vi "Run Tests.vi"(11 "Arguments":string[](array[string])) -> (2 "CLI Message":string, 3 "CLI Return Code":i32)   [LabVIEW 2026]
doc: "Caraya suite runner, generated by lvai_generate_caraya_test_runner.\n\nIt builds every test VI's path relative to its OWN location, so the suite moves with the folder, and runs them through Caraya's Run Tests.vi (Array Path instance) with Interactive FALSE - a TRUE there opens a modal report dialog, which stops LabVIEW's gRPC service until a human dismisses it.\n\nRead the JUnit report named by 'Report Path used', not 'error out': the error cluster carries the FIRST failed assertion only."
uses:
  <vilib>/addons/_JKI Toolkits/Caraya/run-tests/Run Test (Array Path).vi
  <vilib>/addons/_JKI Toolkits/Caraya/Caraya.lvlib
panel:
  out "error out":errorcluster
  out "Report Path used":path
  in  "error in":errorcluster
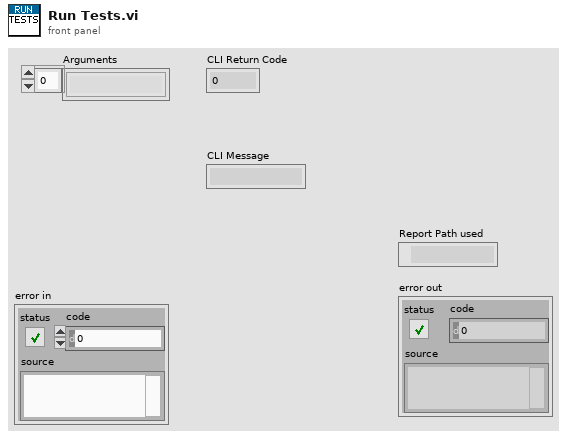
[diagram p1: front panel]
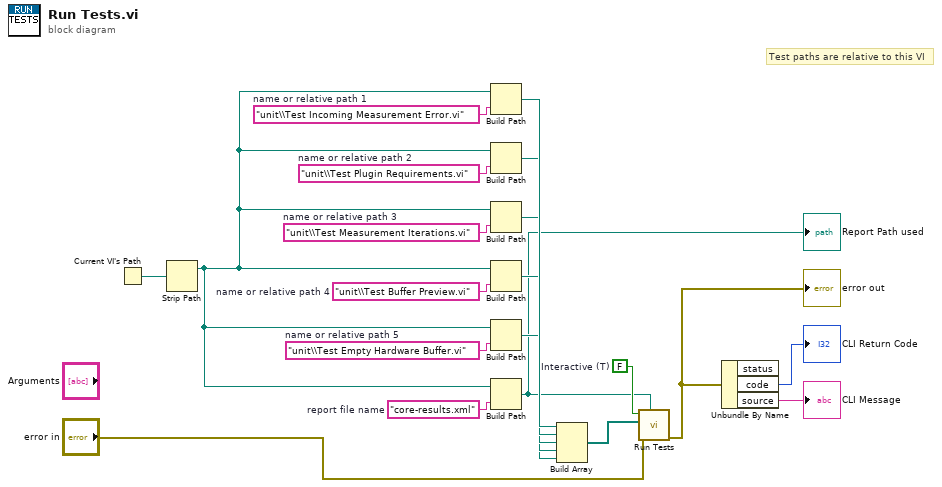
[diagram p0: block diagram]
diagram:
  w7 = FALSE  # Interactive (T)
  w13 = "core-results.xml"  # report file name
  w15 = "unit\\Test Empty Hardware Buffer.vi"  # name or relative path 5
  w16 = "unit\\Test Buffer Preview.vi"  # name or relative path 4
  w17 = "unit\\Test Measurement Iterations.vi"  # name or relative path 3
  w18 = "unit\\Test Plugin Requirements.vi"  # name or relative path 2
  w19 = "unit\\Test Incoming Measurement Error.vi"  # name or relative path 1
  # "Test paths are relative to this VI"
  n1 = Current VI's Path() -> (path=w20:path)
  n2 = Strip Path(path=w20) -> (stripped path=w14:path)  [unwired: 1 out]
  n3 = Build Path(base path=w14, name or relative path=w19) -> (appended path=w12:path)
  n4 = Build Path(base path=w14, name or relative path=w18) -> (appended path=w11:path)
  n5 = Build Path(base path=w14, name or relative path=w17) -> (appended path=w10:path)
  n6 = Build Path(base path=w14, name or relative path=w16) -> (appended path=w9:path)
  n7 = Build Path(base path=w14, name or relative path=w15) -> (appended path=w8:path)
  n8 = Build Path(base path=w14, name or relative path=w13) -> (appended path=w4:path)
  "Report Path used" <- w4
  n9 = Build Array(w12, w11, w10, w9, w8) -> (w6:path[])
  n10 = call-poly <vilib>:"Run Tests.vi"("Report Path"=w4, "error in"="error in", "Paths"=w6, "Interactive (T)"=w7) -> ("error out"=w3:errorcluster)  [unwired: 6 in, 1 out]
  "error out" <- w3
  n11 = Unbundle By Name(w3) -> ("code"=→"CLI Return Code":i32, "source"=→"CLI Message":string)  [unwired: 1 out]
